vi "CSM - Create CSM Palette at Root.vi"() -> ()   [LabVIEW 2017]
doc: "Create a CSM module palette at the root of the function palette."
uses:
  _Shared/CSM Shared.lvlib
  _ui/csm-ui-support.lvlib
panel:
  in  "Remove Button":bool
  in  "Add Button":bool
  out "String":string
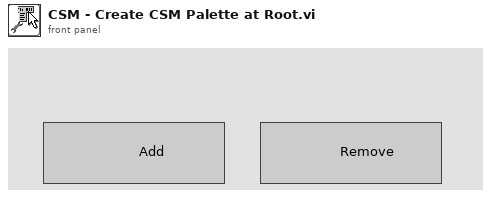
[diagram p1: front panel]
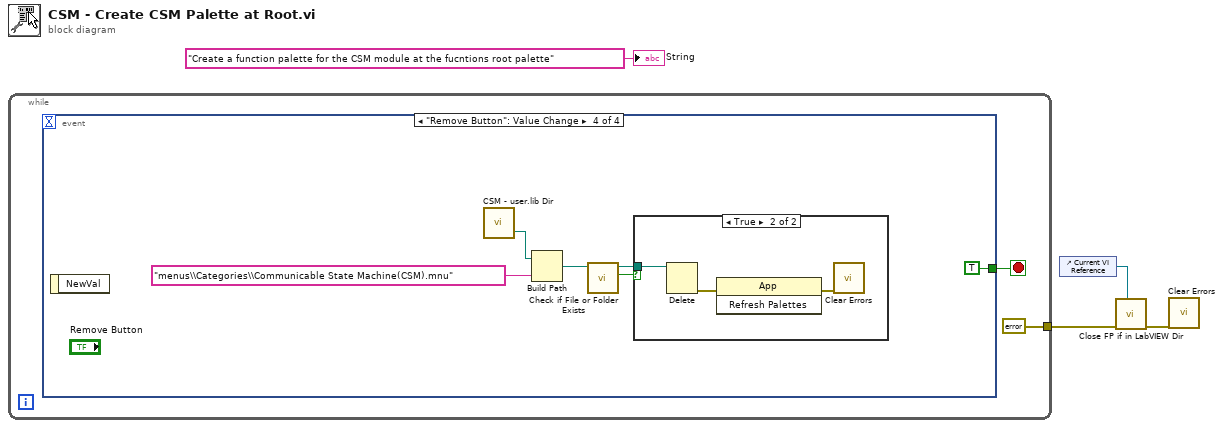
[diagram p0: block diagram]
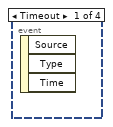
[diagram p2: hidden frame]
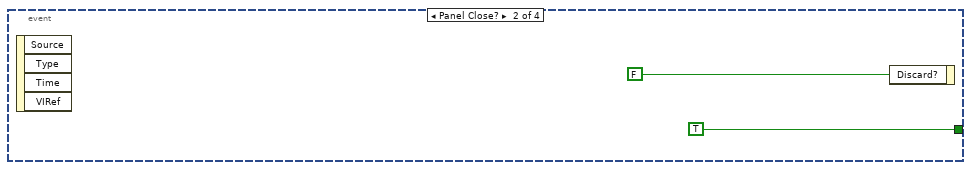
[diagram p3: hidden frame]
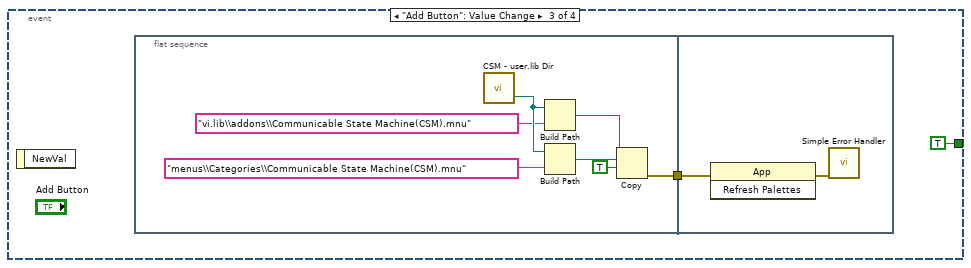
[diagram p4: hidden frame]
diagram:
  n1 = while {
    tunnel: [errorcluster {"status"=FALSE, "code"=0, "source"=""} ("Error in")] -> w1
    stop <- w6 stop-if-true
    n2 = event shown="[3] \"Remove Button\": Value Change" {
      selector: _ -> [_ _ _ _]
      dyn-events: _ -> [_ _ _ _]
      timeout: _ -> [_ _ _ _]
      tunnel: [_ TRUE ("Discard?") TRUE ("Discard?") TRUE ("Discard?")] -> w6
      event Timeout {
        n3 = event-data() -> ()  [unwired: 1 in, 3 out]
      }
      event Panel Close? {
        n4 = event-data() -> ()  [unwired: 1 in, 4 out]
        n5 = event-data("Discard?"=FALSE) -> ()  [unwired: 1 in, 1 out]
      }
      event "Add Button": Value Change {
        n6 = event-data() -> ()  [unwired: 1 in, 1 out]
        n7 = flat-sequence {
          tunnel: [w11] -> w10
          tunnel: w10 -> [w19]
          frame #0 {
            n8 = call "CSM - user.lib Dir.vi"() -> ("<LabVIEW>"=w17:path)  [unwired: 2 in, 1 out]
            n9 = Build Path(base path=w17, name or relative path="vi.lib\\addons\\Communicable State Machine(CSM).mnu") -> (appended path=w14:path)
            n10 = Build Path(base path=w17, name or relative path="menus\\Categories\\Communicable State Machine(CSM).mnu") -> (appended path=w13:path)
            n11 = Copy(9:TRUE ("overwrite (F)"), 10:w13, 11:w14) -> (0:w11:errorcluster)  [unwired: 2 in, 2 out]
          }
          frame #1 {
            n12 = invoke class="App" method="Refresh Palettes"(error in=w19) -> (error out=w18:errorcluster)  [unwired: 2 in, 2 out]
            n13 = call <vilib>:"Simple Error Handler.vi"("error in (no error)"=w18) -> ()  [unwired: 4 in, 5 out]
          }
        }
      }
      event "Remove Button": Value Change {
        n14 = event-data() -> ()  [unwired: 1 in, 1 out]
        n15 = call "CSM - user.lib Dir.vi"() -> ("<LabVIEW>"=w24:path)  [unwired: 2 in, 1 out]
        n16 = Build Path(base path=w24, name or relative path="menus\\Categories\\Communicable State Machine(CSM).mnu") -> (appended path=w21:path)
        n17 = call <vilib>:"Check if File or Folder Exists.vi"("path"=w21) -> ("file or folder exists?"=w23:bool, "dup path"=w22:path)  [unwired: 8 in, 1 out]
        n18 = case shown="True" w23 {
          tunnel: w22 -> [_ w27]
          frame False {
          }
          frame True {
            n19 = Delete(path (use dialog)=w27) -> (error out=w28:errorcluster)  [unwired: 4 in, 2 out]
            n20 = invoke class="App" method="Refresh Palettes"(error in=w28) -> (error out=w26:errorcluster)  [unwired: 2 in, 2 out]
            n21 = call <vilib>:"Clear Errors.vi"("error in (no error)"=w26) -> ()  [unwired: 5 in, 2 out]
          }
        }
      }
    }
  }
  n22 = control-ref of="Current VI Reference"() -> (w2:refnum<vi>)
  n23 = call "Close FP if in LabVIEW Dir.vi"("VI Refnum"=w2, "Error in"=w1) -> ("Error out"=w3:errorcluster)  [unwired: 9 in]
  n24 = call <vilib>:"Clear Errors.vi"("error in (no error)"=w3) -> ()  [unwired: 5 in, 2 out]
  "String" <- "Create a function palette for the CSM module at the fucntions root palette" ("String")
